vi "check if subpanel should be closed.vi"(8 "error in":errorcluster, 10 "SubPanel in":refnum<vi>, 11 "node in":T1) -> (0 "error out":errorcluster, 2 "needs closing":bool, 3 "node out":T1)   [LabVIEW 2013, in "Standard Editor.lvlib"]
uses:
  Standard Editor.lvlib
  <vilib>/NI/Configuration Framework/Node/NodeRef.ctl
  <vilib>/NI/Configuration Framework/Node/NISE_CEF_Node.lvclass
  <vilib>/NI/Configuration Framework/Node/NISE_CEF_Node.lvclass/NISE_CEF_Node.ctl
  <vilib>/NI/Configuration Framework/Node/ReadChildren.vi
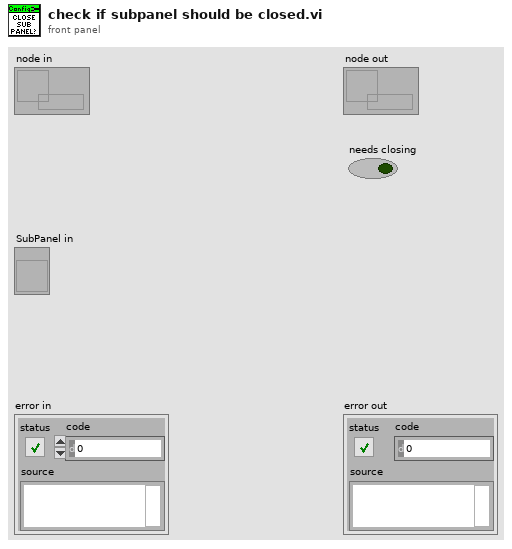
[diagram p1: front panel]
types:
  T1 = typedef "NISE_CEF_Node.lvclass/NodeRef.ctl" = refnum<data-value>
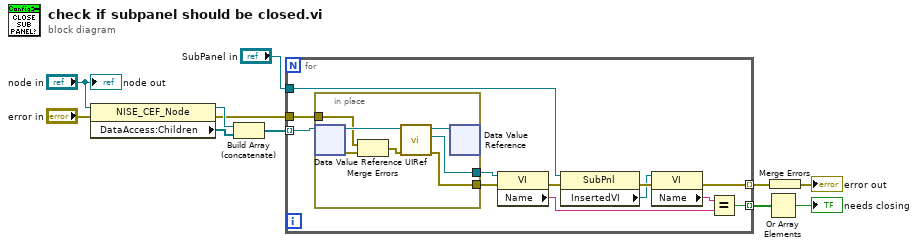
[diagram p0: block diagram]
diagram:
  n1 = property class="NISE_CEF_Node"(reference="node in", error in="error in") -> (reference out=w8:T1, error out=w6:errorcluster, "DataAccess:Children"=w4:T1[])
  n2 = Build Array (concatenate)(w8, w4) -> (w5:T1[])
  n3 = for {
    tunnel: "SubPanel in" -> [w21]
    tunnel: [w17] -> w3 mode=indexing
    tunnel: [w14] -> w10 mode=indexing
    tunnel: w6 -> [w13]
    tunnel: w5 -> [w12] mode=indexing
    n4 = in-place {
      in-place-border: w13 -> [w27]
      in-place-border: [w28] -> w23
      in-place-border: [w26] -> w22
      n5 = in-place-dvr #1(w12) -> (w30:refnum<class "NISE_CEF_Node.lvclass">, w24:errorcluster)
      n6 = Merge Errors(w27, w24) -> (w25:errorcluster)
      n7 = call-dynamic "UIRef.vi"("error in"=w25, "node in"=w30) -> ("error out"=w26:errorcluster, "VI refnum"=w28:refnum<vi>, "node out"=w29:refnum<class "NISE_CEF_Node.lvclass">)  [unwired: 7 in]
      n8 = in-place-dvr #1(w29) -> ()  [unwired: 2 out]
    }
    n9 = property class="VI"(reference=w23, error in=w22) -> (error out=w18:errorcluster, "Name"=w15:string)  [unwired: 1 out]
    n10 = property class="SubPnl"(reference=w21, error in=w18) -> (error out=w20:errorcluster, "InsertedVI"=w19:refnum<vi>)  [unwired: 1 out]
    n11 = property class="VI"(reference=w19, error in=w20) -> (error out=w17:errorcluster, "Name"=w16:string)  [unwired: 1 out]
    n12 = Equal?(x=w16, y=w15) -> (x = y?=w14:bool)
  }
  n13 = Or Array Elements(Boolean array=w10) -> (logical OR=→"needs closing":bool)
  n14 = Merge Errors(w3) -> (→"error out":errorcluster)
  "node out" <- "node in"
